vi "Test Get Account.vi"() -> ()   [LabVIEW 2026]
doc: "Caraya unit test for Get Account.vi (which reads the file with Read Accounts.vi and looks the number up with Find Account.vi). Every case reads its own fresh copy of the specification accounts file (Create Accounts Fixture.vi, written under Tests\\results), so the result does not depend on balances changed by running the ATM.\n\nCase 1: account 23456 is found with its full record from the file.\nCase 2: the unknown account 00000 is not found, and that is not an error (code 0).\n\nThe error cluster carries the FIRST failure only. Read the JUnit report for all of them."
uses:
  <vilib>/addons/_JKI Toolkits/Caraya/classes/Test/Test.lvclass
  <vilib>/addons/_JKI Toolkits/Caraya/classes/Assert/Assert.lvclass
panel:
  out "error out":errorcluster
  in  "error in":errorcluster
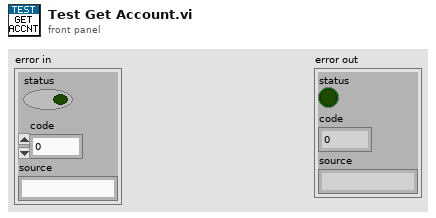
[diagram p1: front panel]
types:
  T1 = cluster{"Account Number":string, "First Name":string, "Last Name":string, "Balance":dbl}
  T2 = typedef "ATM Account.ctl" = cluster{"Account Number":string, "First Name":string, "Last Name":string, "Balance":dbl}
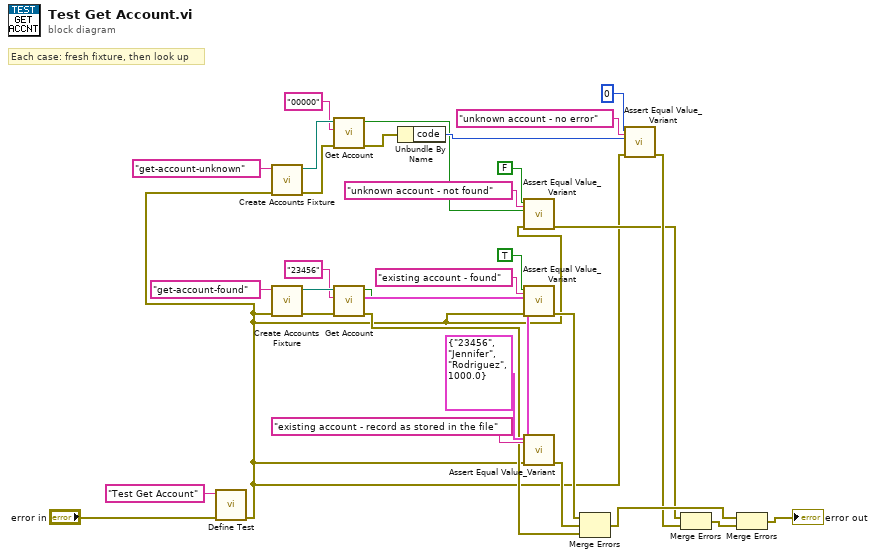
[diagram p0: block diagram]
diagram:
  # "Each case: fresh fixture, then look up"
  n1 = call <vilib>:"Define Test.vi"("error in (no error)"="error in", "Label (VI Title)"="Test Get Account") -> ("error out"=w4:errorcluster)  [unwired: 8 in, 1 out]
  n2 = call "Create Accounts Fixture.vi"("error in"=w4, "Fixture Name"="get-account-unknown") -> ("error out"=w21:errorcluster, "Accounts File Path"=w20:path)  [unwired: 8 in]
  n3 = call "Create Accounts Fixture.vi"("error in"=w4, "Fixture Name"="get-account-found") -> ("error out"=w8:errorcluster, "Accounts File Path"=w7:path)  [unwired: 8 in]
  n4 = call "Get Account.vi"("error in"=w21, "Account Number"="00000", "Accounts File Path"=w20) -> ("error out"=w23:errorcluster, "Account Found?"=w22:bool)  [unwired: 6 in, 1 out]
  n5 = call "Get Account.vi"("error in"=w8, "Account Number"="23456", "Accounts File Path"=w7) -> ("error out"=w11:errorcluster, "Account"=w10:T2, "Account Found?"=w9:bool)  [unwired: 6 in]
  n6 = Unbundle By Name(w23) -> ("code"=w24:i32)
  n7 = call <vilib>:"Assert Equal Value_Variant.vi"("Label"="unknown account - not found", "error in (no error)"=w4, "Actual"=w22, "Expected"=FALSE ("expected 3")) -> ("error out"=w27:errorcluster)  [unwired: 6 in, 1 out]
  n8 = call <vilib>:"Assert Equal Value_Variant.vi"("Label"="existing account - found", "error in (no error)"=w4, "Actual"=w9, "Expected"=TRUE ("expected 1")) -> ("error out"=w14:errorcluster)  [unwired: 6 in, 1 out]
  n9 = call <vilib>:"Assert Equal Value_Variant.vi"("Label"="existing account - record as stored in the file", "error in (no error)"=w4, "Actual"=w10, "Expected"=T1 {"Account Number"="23456", "First Name"="Jennifer", "Last Name"="Rodriguez", "Balance"=1000.0} ("expected 2")) -> ("error out"=w17:errorcluster)  [unwired: 6 in, 1 out]
  n10 = Merge Errors(w14, w17, w11) -> (w31:errorcluster)
  n11 = call <vilib>:"Assert Equal Value_Variant.vi"("Label"="unknown account - no error", "error in (no error)"=w4, "Actual"=w24, "Expected"=0 ("expected 4")) -> ("error out"=w30:errorcluster)  [unwired: 6 in, 1 out]
  n12 = Merge Errors(w27, w30) -> (w32:errorcluster)
  n13 = Merge Errors(w31, w32) -> (→"error out":errorcluster)
